vi "UR LabVIEW Interface.vi"() -> ()   [LabVIEW 2019]
uses:
  Classes/Application/ErrorEvent.ctl
  Classes/Application/Application.lvclass
  Classes/Application/FrontPanelControls.ctl
  Classes/Robot/Universal Robot/Universal Robot.lvclass
  Classes/Robot/UR CB-Series/UR CB-Series.lvclass
  C:/_Code/Development/Sub-Zero Functional Test/standard hardware/Universal Robots/UR LabVIEW Interface/Classes/Robot/Universal Robot/Universal Robot.lvclass
  Classes/Robot/UR E-Series/UR E-Series.lvclass
  Classes/Client Interfaces/Dashboard Server/Dashboard Server.lvclass
  Classes/Client Interfaces/Socket Communication/Socket Communication.lvclass
  Classes/Application/Application Interfaces/Operation Interface/Operation Interface.lvclass
  C:/_Code/Development/Sub-Zero Functional Test/standard hardware/Universal Robots/UR LabVIEW Interface/Classes/Application/Application Interfaces/Application Interface/Application Interface.lvclass
  Classes/Application/Application Interfaces/Command Interface/Command Interface.lvclass
  Classes/Application/Application Interfaces/Program Interface/Program Interface.lvclass
  Classes/Application/Application Interfaces/Socket Auto Connect/Socket Auto Connect.lvclass
  Classes/Application/Application Interfaces/Error Interface/Error Interface.lvclass
  Classes/Application/Application Interfaces/Application Interface/Application Interface.lvclass
panel:
  in  "status":string
  out "Main Header":string
  in  "connect":bool
  out "Polyscope Version":string
  out "Operation Header":string
  out "Program Header":string
  out "Command Header":string
  out "Socket Interface":string
  out "Error Header":string
  in  "abort":bool
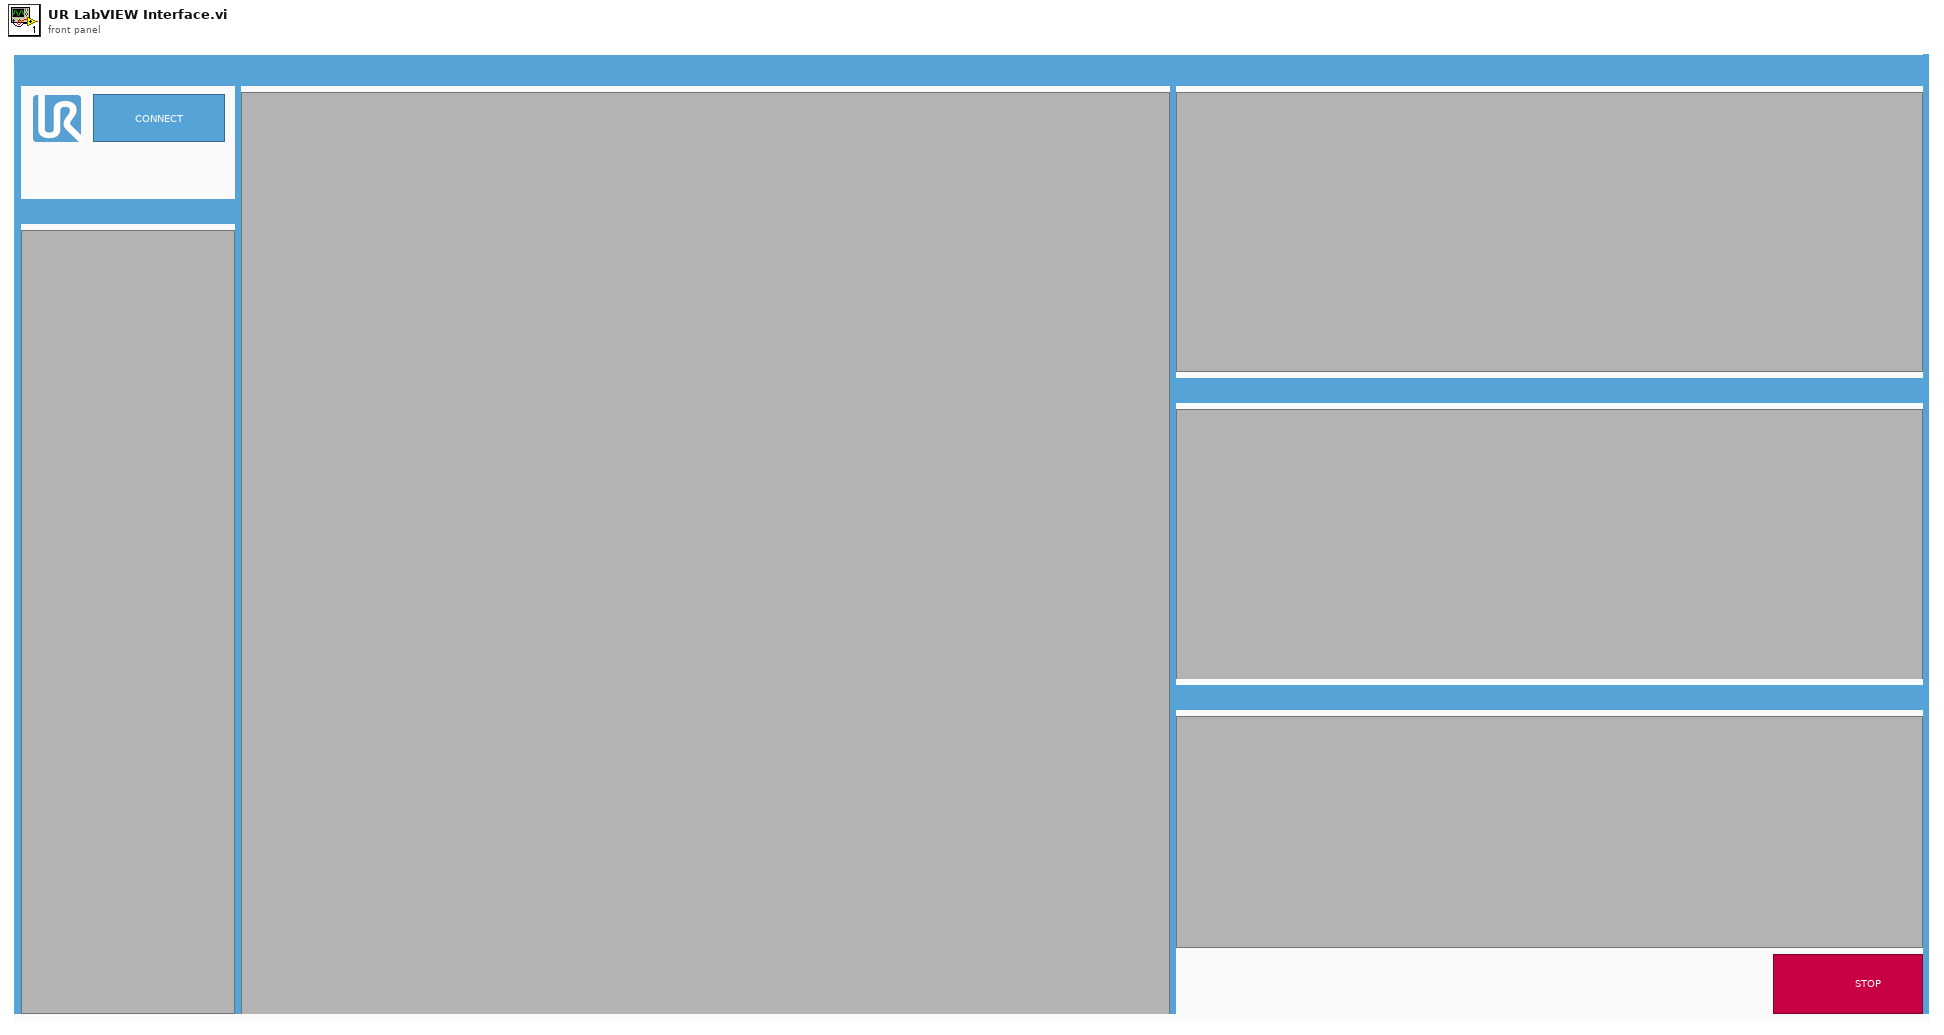
[diagram p1: front panel]
types:
  T1 = typedef "Application.lvclass/ErrorEvent.ctl" = cluster{"VI":string, "Time Stamp":timestamp, "Error":errorcluster, "Fatal":bool}
  T2 = typedef "Application.lvclass/FrontPanelControls.ctl" = cluster{"Operation Interface":refnum<vi>, "Program Interface":refnum<vi>, "Command Interface":refnum<vi>, "Socket Interface":refnum<vi>, "Error Interface":refnum<vi>}
  T3 = typedef "Application.lvclass/ApplicationSettings.ctl" = cluster{"Robot IP":string, "Socket Host IP":string, "Robot Type":T4, "Use SFTP Program List":bool, "Robot Logging":bool, "TCP Logging":bool, "Fault Program":string}
  T4 = typedef "Application.lvclass/RobotType.ctl" = enum16{"UR E-Series", "UR CB-Series"}
  T5 = enum32{"invalid app kind", "Development System", "Run Time System", "Student Edition", "Embedded LabVIEW", "Evaluation", "Custom"}
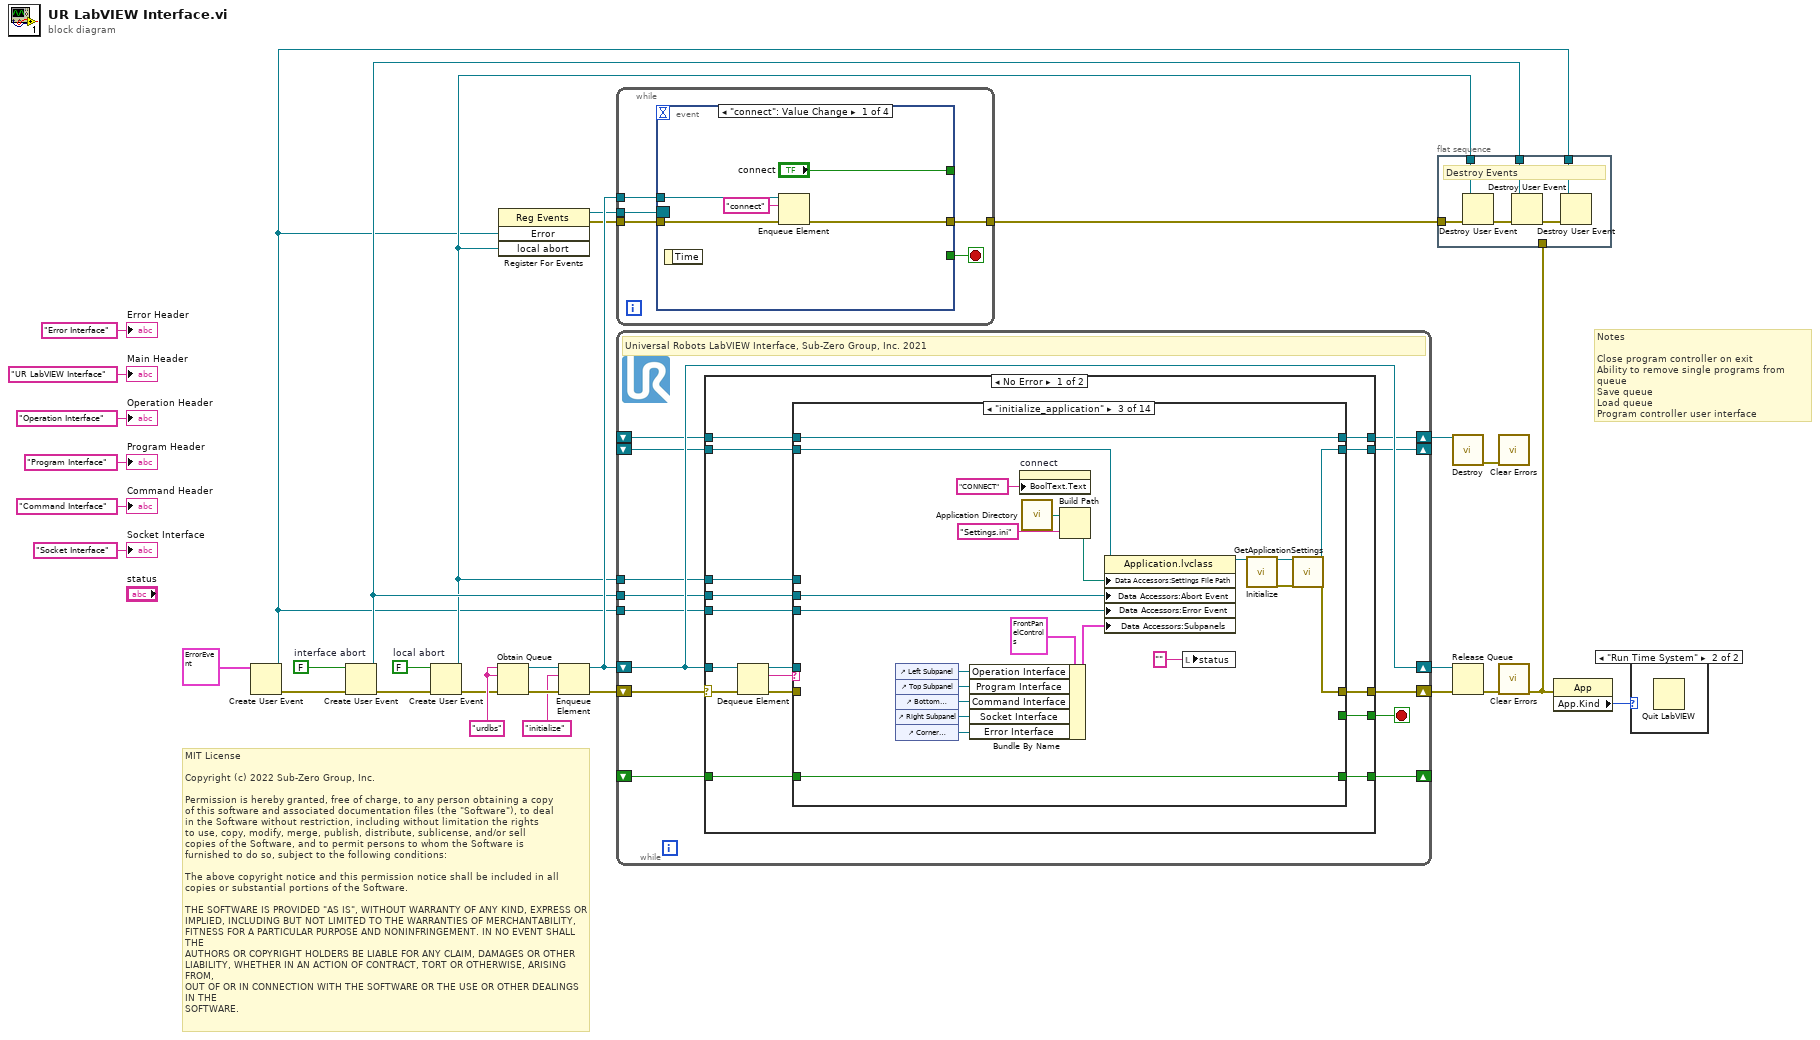
[diagram p0: block diagram]
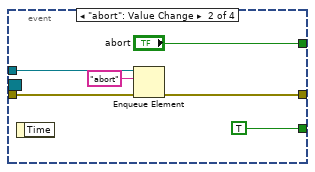
[diagram p3: hidden frame]
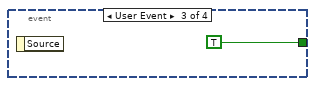
[diagram p4: hidden frame]
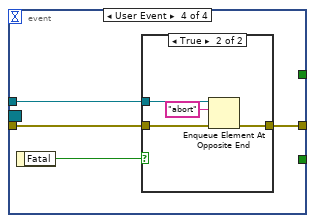
[diagram p5: hidden frame]
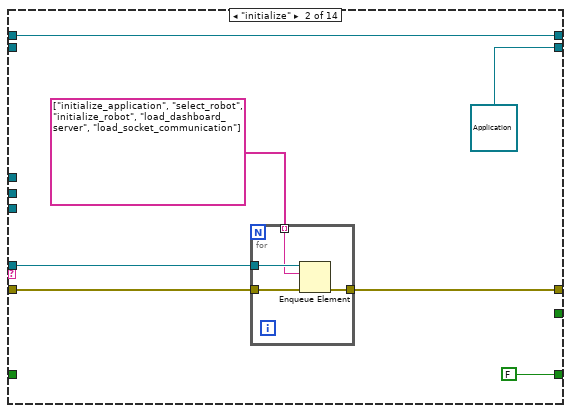
[diagram p8: hidden frame]
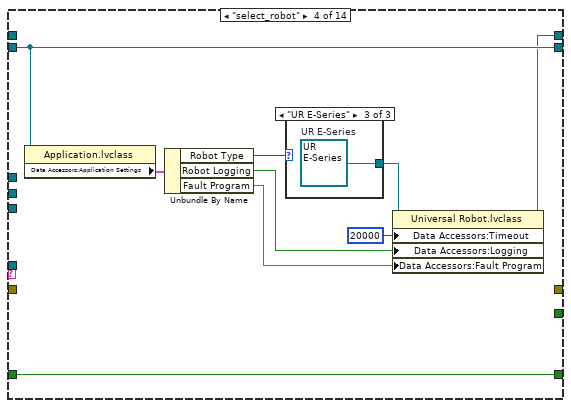
[diagram p9: hidden frame]
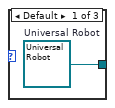
[diagram p10: hidden frame]
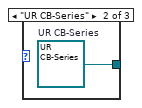
[diagram p11: hidden frame]
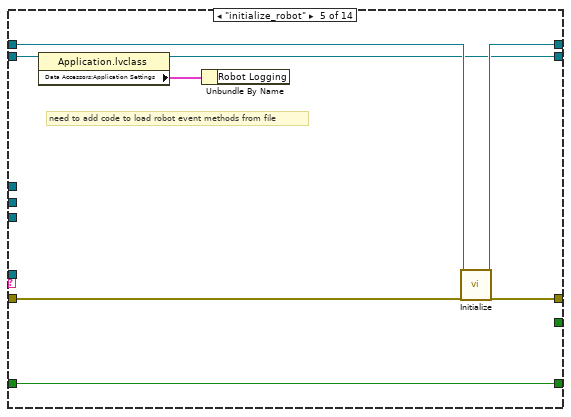
[diagram p12: hidden frame]
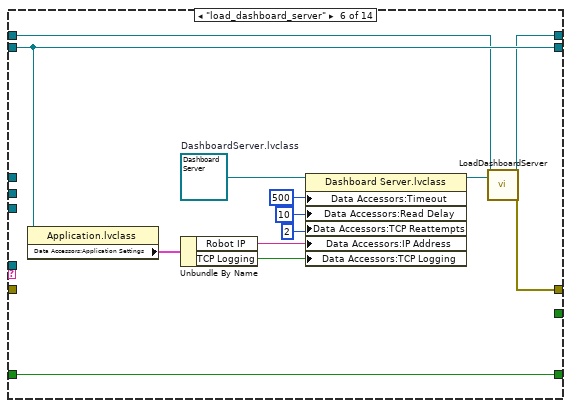
[diagram p13: hidden frame]
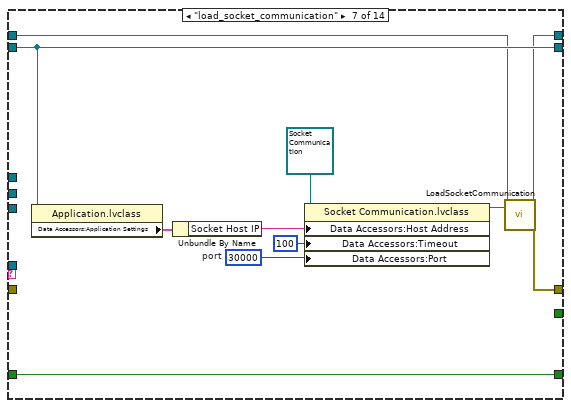
[diagram p14: hidden frame]
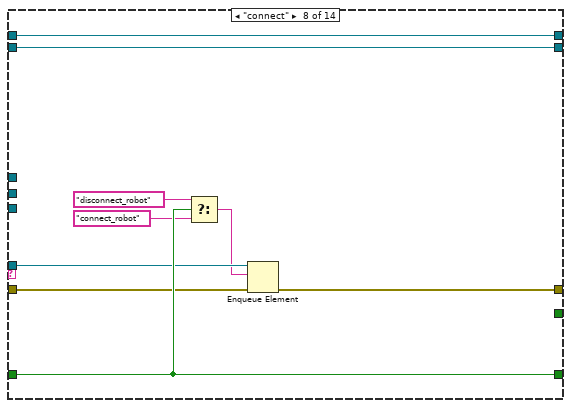
[diagram p15: hidden frame]
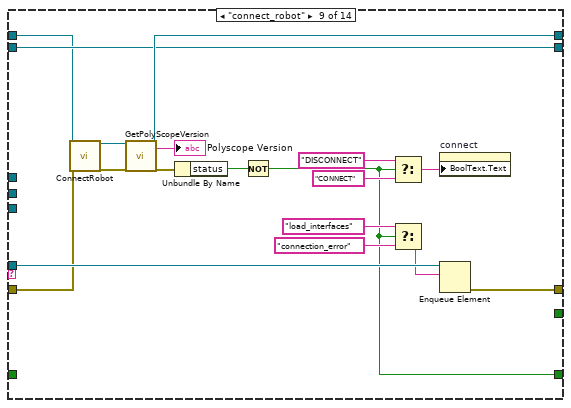
[diagram p16: hidden frame]
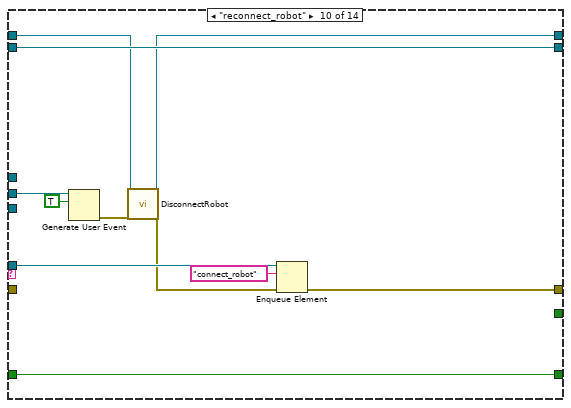
[diagram p17: hidden frame]
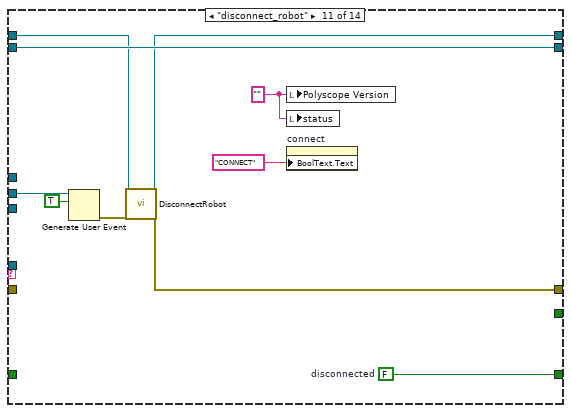
[diagram p18: hidden frame]
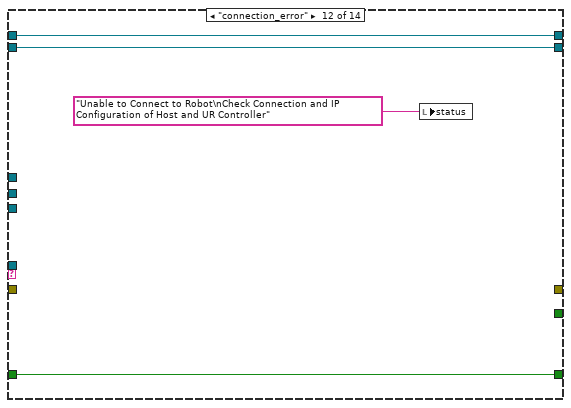
[diagram p19: hidden frame]
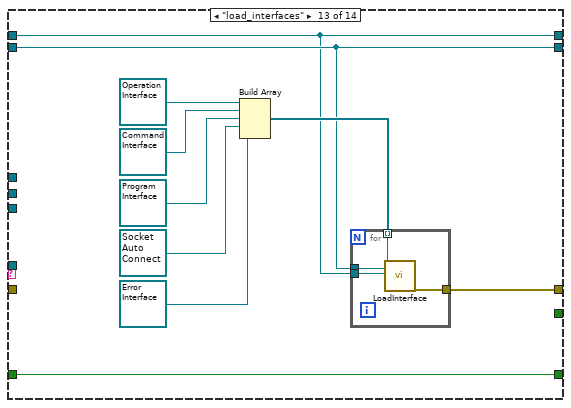
[diagram p20: hidden frame]
diagram:
  w12 = FALSE  # local abort
  w21 = FALSE  # interface abort
  w26 = "urdbs" ("name (unnamed)")
  # "MIT License\n\nCopyright (c) 2022 Sub-Zero Group, Inc.\n\nPermission is hereby granted, free of charge, to any person obtaining a copy\nof this software and associated documentation files (the \"Software\"), to deal\nin the Software without restriction, including without limitation the rights\nto use, copy, modify, merge, publish, distribute, sublicense, and/or sell\ncopies of the Software, and to permit persons to whom the Software is\nfurnished to do so, subject to the following conditions:\n\nThe above copyright notice and this permission notice shall be included in all\ncopies or substantial portions of the Software.\n\nTHE SOFTWARE IS PROVIDED \"AS IS\", WITHOUT WARRANTY OF ANY KIND, EXPRESS OR\nIMPLIED, INCLUDING BUT NOT LIMITED TO THE WARRANTIES OF MERCHANTABILITY,\nFITNESS FOR A PARTICULAR PURPOSE AND NONINFRINGEMENT. IN NO EVENT SHALL THE\nAUTHORS OR COPYRIGHT HOLDERS BE LIABLE FOR ANY CLAIM, DAMAGES OR OTHER\nLIABILITY, WHETHER IN AN ACTION OF CONTRACT, TORT OR OTHERWISE, ARISING FROM,\nOUT OF OR IN CONNECTION WITH THE SOFTWARE OR THE USE OR OTHER DEALINGS IN THE\nSOFTWARE."
  # "Notes\n\nClose program controller on exit\nAbility to remove single programs from queue\nSave queue\nLoad queue\nProgram controller user interface"
  n1 = Create User Event(user event datatype=T1 {"VI"="", "Time Stamp"=timestamp(0 s since 1904-01-01), "Error"={"status"=FALSE, "code"=0, "source"=""}, "Fatal"=FALSE} ("Error")) -> (user event=w9:refnum<user-event>, error out=w20:errorcluster)  [unwired: 1 in]
  n2 = Create User Event(user event datatype=w21, error in=w20) -> (user event=w19:refnum<user-event>, error out=w14:errorcluster)
  n3 = Create User Event(user event datatype=w12, error in=w14) -> (user event=w11:refnum<user-event>, error out=w13:errorcluster)
  n4 = Obtain Queue(name (unnamed)=w26, element data type=w26, error in (no error)=w13) -> (queue out=w30:refnum<queue>, error out=w31:errorcluster)  [unwired: 2 in, 1 out]
  n5 = register-events(w9, w11) -> (reference out=w15:refnum<event-registration>, error out=w23:errorcluster)  [unwired: 2 in]
  n6 = Enqueue Element(queue=w30, element="initialize", error in (no error)=w31) -> (queue out=w27:refnum<queue>, error out=w28:errorcluster)  [unwired: 1 in, 1 out]
  n7 = while {
    tunnel: w27 -> [w36]
    tunnel: w23 -> [w35]
    tunnel: w15 -> [w34]
    tunnel: [w33] -> w22
    stop <- w32 stop-if-true
    n8 = event shown="[0] \"connect\": Value Change" {
      selector: w34 -> [_ _ _ _]
      dyn-events: _ -> [_ _ _ _]
      timeout: _ -> [_ _ _ _]
      tunnel: w36 -> [w41 w47 _ w52]
      tunnel: w35 -> [w40 w46 _ w50]
      tunnel: [w39 w45 _ w51] -> w33
      tunnel: [_ TRUE TRUE _] -> w32
      tunnel: ["connect" "abort" _ _] -> _
      event "connect": Value Change {
        n9 = event-data() -> ()  [unwired: 1 in, 1 out]
        n10 = Enqueue Element(queue=w41, element="connect", error in (no error)=w40) -> (error out=w39:errorcluster)  [unwired: 1 in, 2 out]
      }
      event "abort": Value Change {
        n11 = event-data() -> ()  [unwired: 1 in, 1 out]
        n12 = Enqueue Element(queue=w47, element="abort", error in (no error)=w46) -> (error out=w45:errorcluster)  [unwired: 1 in, 2 out]
      }
      event User Event {
        n13 = event-data() -> ()  [unwired: 1 in, 1 out]
      }
      event User Event {
        n14 = event-data() -> ("Fatal"=w49:bool)  [unwired: 1 in]
        n15 = case shown="True" w49 {
          tunnel: w52 -> [_ w57]
          tunnel: [w53 w55] -> w51
          tunnel: w50 -> [w53 w56]
          frame False {
          }
          frame True {
            n16 = Enqueue Element At Opposite End(queue=w57, element="abort", error in (no error)=w56) -> (error out=w55:errorcluster)  [unwired: 1 in, 2 out]
          }
        }
      }
    }
  }
  n17 = while {
    shift-right: [w68] -> w24
    shift-left: w28 -> [w70]
    shift-right: [w69] -> w25
    shift-left: w27 -> [w69]
    tunnel: w19 -> [w67]
    shift-right: [w65] -> w18
    shift-left: _ -> [w64]
    shift-right: [w63] -> _
    shift-left: _ -> [w62]
    tunnel: w9 -> [w61]
    shift-right: [w60] -> _
    shift-left: _ -> [w59]
    tunnel: w11 -> [w58]
    stop <- w66 stop-if-true
    # "Universal Robots LabVIEW Interface, Sub-Zero Group, Inc. 2021"
    n18 = case shown="No Error" w70 {
      selector: w70 -> [w85 w243]
      tunnel: w69 -> [w86 _]
      tunnel: [w81 _] -> w68
      tunnel: w67 -> [w75 _]
      tunnel: [w80 _] -> w66
      tunnel: [w79 w245] -> w65
      tunnel: w64 -> [w78 w245]
      tunnel: [w77 w242] -> w63
      tunnel: w62 -> [w76 w242]
      tunnel: w61 -> [w74 _]
      tunnel: [w73 w244] -> w60
      tunnel: w59 -> [w72 w244]
      tunnel: w58 -> [w71 _]
      frame No Error {
        n19 = Dequeue Element(queue=w86, error in (no error)=w85) -> (queue out=w82:refnum<queue>, element=w83:string, error out=w84:errorcluster)  [unwired: 1 in, 1 out]
        n20 = case shown="\"initialize_application\"" w83 {
          tunnel: w84 -> [w90 w97 _ _ w137 _ _ w172 w180 _ _ _ _ w234]
          tunnel: w82 -> [_ w96 _ _ _ _ _ w173 w191 w201 _ _ _ _]
          tunnel: [w90 w95 w106 _ w141 w147 w158 w171 w190 w199 w209 _ w222 w234] -> w81
          tunnel: [_ _ _ _ _ _ _ _ _ _ _ _ _ TRUE] -> w80
          tunnel: [w89 w91 w123 w127 w142 w148 w159 w176 w194 w202 w213 w219 w225 w240] -> w79
          tunnel: w78 -> [w89 w91 w123 _ w138 w149 w160 w176 w183 w203 w214 w219 w225 w240]
          tunnel: [w88 refnum<class "Application.lvclass"> refnum ("Application.lvclass") w107 w131 w136 w152 w166 w175 w192 w205 w215 w218 w226 w239] -> w77
          tunnel: w76 -> [w88 _ w110 w131 w140 w152 w166 w175 w192 w205 w215 w218 w226 w239]
          tunnel: w75 -> [_ _ w118 _ _ _ _ _ _ w197 w212 _ _ w238]
          tunnel: w74 -> [_ _ w102 _ _ _ _ _ _ _ _ _ _ _]
          tunnel: [w87 FALSE ("connected") w116 w132 w143 w153 w167 w174 w177 w204 w206 w217 w229 w237] -> w73
          tunnel: w72 -> [w87 _ w116 w132 w143 w153 w167 w174 _ w204 _ w217 w229 w237]
          tunnel: w71 -> [_ _ _ _ _ _ _ _ _ _ _ _ _ w236]
          frame Default {
          }
          frame "initialize" {
            n21 = for {
              tunnel: w97 -> [w101]
              tunnel: w96 -> [w100]
              tunnel: [w99] -> w95
              tunnel: string[] ["initialize_application", "select_robot", "initialize_robot", "load_dashboard_server", "load_socket_communication"] -> [w98] mode=indexing
              n22 = Enqueue Element(queue=w100, element=w98, error in (no error)=w101) -> (error out=w99:errorcluster)  [unwired: 1 in, 2 out]
            }
          }
          frame "initialize_application" {
            n23 = control-ref of="Left Subpanel"() -> (w121:refnum<vi>)
            n24 = control-ref of="Top Subpanel"() -> (w120:refnum<vi>)
            n25 = control-ref of="Bottom Subpanel"() -> (w119:refnum<vi>)
            n26 = control-ref of="Right Subpanel"() -> (w104:refnum<vi>)
            n27 = control-ref of="Corner Subpanel"() -> (w103:refnum<vi>)
            n28 = Bundle By Name(cluster=T2 {"Operation Interface"=refnum, "Program Interface"=refnum, "Command Interface"=refnum, "Socket Interface"=refnum, "Error Interface"=refnum} ("frontPanelControls"), "Operation Interface"=w121, "Program Interface"=w120, "Command Interface"=w119, "Socket Interface"=w104, "Error Interface"=w103) -> (w117:T2)
            n29 = property on="connect" class="Bool"("BoolText.Text"="CONNECT" ("Boolean Text.Text")) -> ()  [unwired: 2 in, 2 out]
            n30 = call <vilib>:"Application Directory.vi"() -> ("Application Directory"=w112:path)
            n31 = Build Path(base path=w112, name or relative path="Settings.ini") -> (appended path=w113:path)
            n32 = property class="Application.lvclass"(reference=w110, "Data Accessors:Settings File Path"=w113, "Data Accessors:Abort Event"=w118, "Data Accessors:Error Event"=w102, "Data Accessors:Subpanels"=w117) -> (reference out=w114:refnum<class "Application.lvclass">)  [unwired: 1 in, 1 out]
            n33 = local write "status"("" ("status")) -> ()
            n34 = call-dynamic "Initialize.vi"("Application in"=w114) -> ("Application out"=w109:refnum<class "Application.lvclass">, "error out"=w108:errorcluster)  [unwired: 17 in]
            n35 = call-dynamic "GetApplicationSettings.vi"("Application in"=w109, "error in (no error)"=w108) -> ("Application out"=w107:refnum<class "Application.lvclass">, "error out"=w106:errorcluster)  [unwired: 16 in]
          }
          frame "select_robot" {
            n36 = property class="Application.lvclass"(reference=w131) -> ("Data Accessors:Application Settings"=w130:T3)  [unwired: 1 in, 2 out]
            n37 = Unbundle By Name(w130) -> ("Robot Type"=w129:T4, "Robot Logging"=w124:bool, "Fault Program"=w125:string)
            n38 = case shown="\"UR E-Series\"" w129 {
              tunnel: [w133 w134 w135] -> w128
              frame Default {
                w133 = refnum<class "Universal Robot.lvclass"> refnum  # Universal Robot
              }
              frame "UR CB-Series" {
                w134 = refnum<class "UR CB-Series.lvclass"> refnum  # UR CB-Series
              }
              frame "UR E-Series" {
                w135 = refnum<class "UR E-Series.lvclass"> refnum  # UR E-Series
              }
            }
            n39 = property class="Universal Robot.lvclass"(reference=w128, "Data Accessors:Timeout"=u32 20000 ("Timeout"), "Data Accessors:Logging"=w124, "Data Accessors:Fault Program"=w125) -> (reference out=w127:refnum<class "Universal Robot.lvclass">)  [unwired: 1 in, 1 out]
          }
          frame "initialize_robot" {
            # "need to add code to load robot event methods from file"
            n40 = property class="Application.lvclass"(reference=w140) -> (reference out=w136:refnum<class "Application.lvclass">, "Data Accessors:Application Settings"=w139:T3)  [unwired: 1 in, 1 out]
            n41 = Unbundle By Name(w139) -> ()  [unwired: 1 out]
            n42 = call-dynamic "Initialize.vi"("Universal Robot in"=w138, "error in (no error)"=w137) -> ("Universal Robot out"=w142:refnum<class "Universal Robot.lvclass">, "error out"=w141:errorcluster)  [unwired: 16 in]
          }
          frame "load_dashboard_server" {
            w156 = refnum<class "Dashboard Server.lvclass"> refnum  # DashboardServer.lvclass
            n43 = property class="Application.lvclass"(reference=w152) -> ("Data Accessors:Application Settings"=w151:T3)  [unwired: 1 in, 2 out]
            n44 = Unbundle By Name(w151) -> ("Robot IP"=w145:string, "TCP Logging"=w144:bool)
            n45 = property class="Dashboard Server.lvclass"(reference=w156, "Data Accessors:Timeout"=500 ("timeout"), "Data Accessors:Read Delay"=u32 10 ("readDelay"), "Data Accessors:TCP Reattempts"=2 ("TCP Reattempts"), "Data Accessors:IP Address"=w145, "Data Accessors:TCP Logging"=w144) -> (reference out=w150:refnum<class "Dashboard Server.lvclass">)  [unwired: 1 in, 1 out]
            n46 = call-dynamic "LoadDashboardServer.vi"("Universal Robot in"=w149, "DashboardServer"=w150) -> ("Universal Robot out"=w148:refnum<class "Universal Robot.lvclass">, "error out"=w147:errorcluster)  [unwired: 16 in]
          }
          frame "load_socket_communication" {
            w157 = u16 30000  # port
            n47 = property class="Application.lvclass"(reference=w166) -> ("Data Accessors:Application Settings"=w165:T3)  [unwired: 1 in, 2 out]
            n48 = Unbundle By Name(w165) -> ("Socket Host IP"=w164:string)
            n49 = property class="Socket Communication.lvclass"(reference=refnum<class "Socket Communication.lvclass"> refnum ("TCP Socket.lvclass"), "Data Accessors:Host Address"=w164, "Data Accessors:Timeout"=100 ("Timeout"), "Data Accessors:Port"=w157) -> (reference out=w161:refnum<class "Socket Communication.lvclass">)  [unwired: 1 in, 1 out]
            n50 = call-dynamic "LoadSocketCommunication.vi"("Universal Robot in"=w160, "Socket Communication"=w161) -> ("Universal Robot out"=w159:refnum<class "Universal Robot.lvclass">, "error out"=w158:errorcluster)  [unwired: 16 in]
          }
          frame "connect" {
            n51 = Select(t="disconnect_robot", s=w174, f="connect_robot") -> (s? t:f=w168:string)
            n52 = Enqueue Element(queue=w173, element=w168, error in (no error)=w172) -> (error out=w171:errorcluster)  [unwired: 1 in, 2 out]
          }
          frame "connect_robot" {
            n53 = call-dynamic "ConnectRobot.vi"("Universal Robot.lvclass in"=w183, "error in (no error)"=w180) -> ("Universal Robot.lvclass out"=w182:refnum<class "Universal Robot.lvclass">, "error out"=w181:errorcluster)  [unwired: 16 in]
            n54 = call-dynamic "GetPolyScopeVersion.vi"("Universal Robot.lvclass in"=w182, "error in (no error)"=w181) -> ("Universal Robot.lvclass out"=w194:refnum<class "Universal Robot.lvclass">, "polyscopeVersion"=→"Polyscope Version":string, "error out"=w179:errorcluster)  [unwired: 15 in]
            n55 = Unbundle By Name(w179) -> ("status"=w178:bool)
            n56 = Not(x=w178) -> (.not. x?=w177:bool)
            n57 = Select(t="DISCONNECT" ("Boolean Text.Text"), s=w177, f="CONNECT" ("Boolean Text.Text")) -> (s? t:f=w184:string)
            n58 = Select(t="load_interfaces", s=w177, f="connection_error") -> (s? t:f=w188:string)
            n59 = property on="connect" class="Bool"("BoolText.Text"=w184) -> ()  [unwired: 2 in, 2 out]
            n60 = Enqueue Element(queue=w191, element=w188) -> (error out=w190:errorcluster)  [unwired: 2 in, 2 out]
          }
          frame "reconnect_robot" {
            n61 = Generate User Event(user event=w197, event data cluster=TRUE ("event data")) -> (error out=w195:errorcluster)  [unwired: 2 in, 1 out]
            n62 = call-dynamic "DisconnectRobot.vi"("Universal Robot.lvclass in"=w203, "error in (no error)"=w195) -> ("Universal Robot.lvclass out"=w202:refnum<class "Universal Robot.lvclass">, "error out"=w200:errorcluster)  [unwired: 16 in]
            n63 = Enqueue Element(queue=w201, element="connect_robot", error in (no error)=w200) -> (error out=w199:errorcluster)  [unwired: 1 in, 2 out]
          }
          frame "disconnect_robot" {
            w206 = FALSE  # disconnected
            w208 = "" ("polyscopeVersion")
            n64 = Generate User Event(user event=w212, event data cluster=TRUE ("event data")) -> (error out=w210:errorcluster)  [unwired: 2 in, 1 out]
            n65 = call-dynamic "DisconnectRobot.vi"("Universal Robot.lvclass in"=w214, "error in (no error)"=w210) -> ("Universal Robot.lvclass out"=w213:refnum<class "Universal Robot.lvclass">, "error out"=w209:errorcluster)  [unwired: 16 in]
            n66 = local write "Polyscope Version"(w208) -> ()
            n67 = local write "status"(w208) -> ()
            n68 = property on="connect" class="Bool"("BoolText.Text"="CONNECT" ("Boolean Text.Text")) -> ()  [unwired: 2 in, 2 out]
          }
          frame "connection_error" {
            n69 = local write "status"("Unable to Connect to Robot\nCheck Connection and IP Configuration of Host and UR Controller" ("status")) -> ()
          }
          frame "load_interfaces" {
            n70 = Build Array(refnum<class "Operation Interface.lvclass"> refnum ("Operation Interface.lvclass"), refnum<class "Command Interface.lvclass"> refnum ("Command Interface.lvclass"), refnum<class "Program Interface.lvclass"> refnum ("Program Interface.lvclass"), refnum<class "Socket Auto Connect.lvclass"> refnum ("Auto Connect TCP Socket Viewer.lvclass"), refnum<class "Error Interface.lvclass"> refnum ("Error Interface.lvclass")) -> (w227:refnum<class "Application Interface.lvclass">[])
            n71 = for {
              tunnel: w227 -> [w233] mode=indexing
              tunnel: w226 -> [w232]
              tunnel: w225 -> [w231]
              tunnel: [w230] -> w222
              n72 = call "LoadInterface.vi"("Application Interface in"=w233, "application"=w232, "universalRobot"=w231) -> ("error out"=w230:errorcluster)  [unwired: 15 in, 1 out]
            }
          }
          frame "abort" {
            w235 = TRUE ("event data")
            n73 = Generate User Event(user event=w238, event data cluster=w235) -> ()  [unwired: 2 in, 2 out]
            n74 = Generate User Event(user event=w236, event data cluster=w235) -> ()  [unwired: 2 in, 2 out]
          }
        }
      }
      frame Error {
        n75 = call "Generate Error.vi"("Application in"=w242, "error in (no error)"=w243) -> ()  [unwired: 17 in, 1 out]
      }
    }
  }
  n76 = flat-sequence {
    tunnel: w22 -> [w248]
    tunnel: w19 -> [w251]
    tunnel: w9 -> [w249]
    tunnel: w11 -> [w246]
    tunnel: w7 -> [_]
    frame #0 {
      # "Destroy Events"
      n77 = Destroy User Event(user event=w246, error in=w248) -> (error out=w247:errorcluster)
      n78 = Destroy User Event(user event=w251, error in=w247) -> (error out=w250:errorcluster)
      n79 = Destroy User Event(user event=w249, error in=w250) -> ()  [unwired: 1 out]
    }
  }
  n80 = call-dynamic "Destroy.vi"("Universal Robot in"=w18) -> ("error out"=w8:errorcluster)  [unwired: 17 in, 1 out]
  n81 = Release Queue(queue=w25, error in (no error)=w24) -> (error out=w16:errorcluster)  [unwired: 1 in, 2 out]
  n82 = call <vilib>:"Clear Errors.vi"("error in (no error)"=w8) -> ()  [unwired: 5 in, 2 out]
  n83 = call <vilib>:"Clear Errors.vi"("error in (no error)"=w16) -> ("error out"=w7:errorcluster)  [unwired: 5 in, 1 out]
  n84 = property class="App"(error in=w7) -> ("App.Kind"=w17:T5)  [unwired: 1 in, 2 out]
  n85 = case shown="\"Run Time System\"" w17 {
    frame Default {
    }
    frame "Run Time System" {
      n86 = Quit LabVIEW() -> ()  [unwired: 1 in]
    }
  }
  "Operation Header" <- "Operation Interface" ("Command Interface Header")
  "Program Header" <- "Program Interface" ("Program Header")
  "Command Header" <- "Command Interface" ("Command Header")
  "Main Header" <- "UR LabVIEW Interface" ("Main Header")
  "Error Header" <- "Error Interface" ("Command Interface Header 6")
  "Socket Interface" <- "Socket Interface" ("Socket Interface")
